vi "test_client.vi"() -> ()   [LabVIEW 2020]
uses:
  Client/Client.lvclass
  Request/Request.lvclass
  ClientBuilder/ClientBuilder.lvclass
  RequestBuilder/RequestBuilder.lvclass
  Types/http_method_enum.ctl
  reqwest.lvlib
  Headers/Headers.lvclass
panel:
  out "client_builder_error":string
  out "request_builder_error":string
  out "status code":u16
  out "response error":string
  out "has_response_error":bool
  in  "auth token":string
  in  "username":string
  in  "password":string
  out "response header":cluster{"header":string, "value":string}[](array[cluster])
  in  "file":path
  out "is_complete":bool
  out "progress":i32
  in  "abort":bool
  out "success":bool
  out "response body":string
  out "error out":errorcluster
  in  "url":string="https://www.vipm.io"
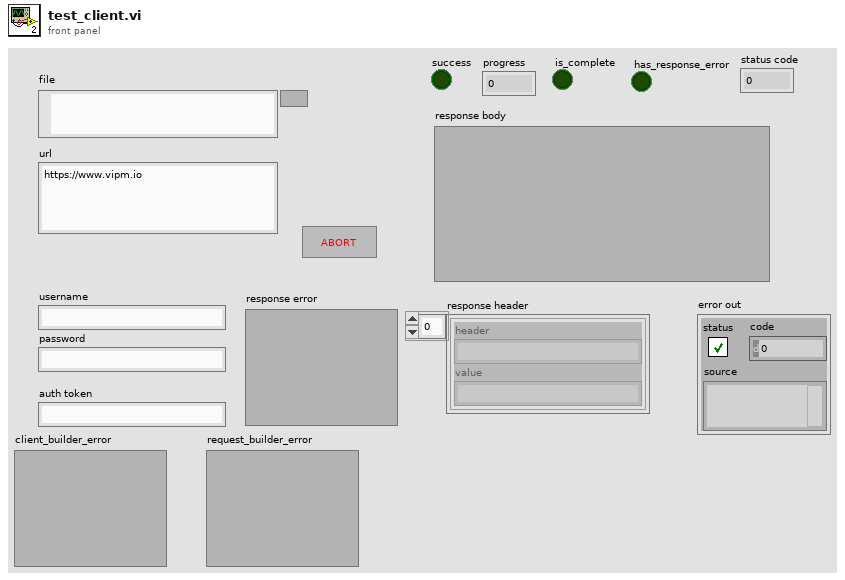
[diagram p1: front panel]
types:
  T1 = typedef "reqwest.lvlib/http_method_enum.ctl" = enum8{"<select>", "GET", "POST", "PUT", "DELETE", "HEAD", "OPTIONS", "CONNECT", "PATCH", "TRACE"}
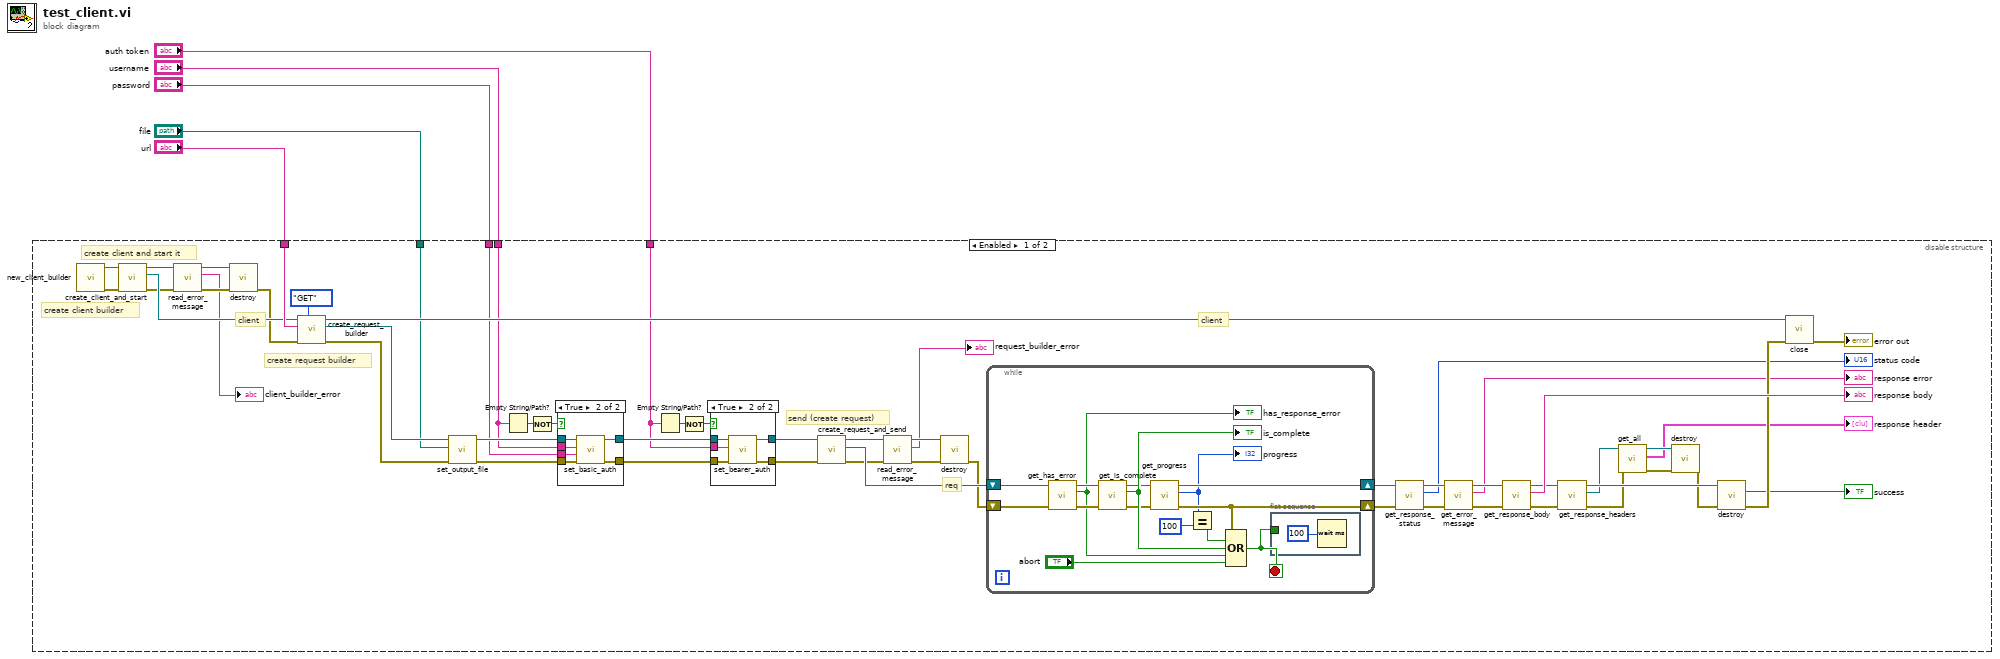
[diagram p0: block diagram]
diagram:
  n1 = disable-structure shown="Enabled" {
    disable-tunnel: "url" -> [w55 _]
    disable-tunnel: "file" -> [w49 _]
    disable-tunnel: "username" -> [w35 _]
    disable-tunnel: "password" -> [w34 _]
    disable-tunnel: "auth token" -> [w29 _]
    frame Enabled {
      # "send (create request)"
      # "create client builder"
      # "client"
      # "create client and start it"
      # "req"
      # "create request builder"
      # "client"
      n2 = call "new_client_builder.vi"() -> ("error out"=w56:errorcluster, "Client out"=w57:refnum<class "ClientBuilder.lvclass">)  [unwired: 10 in]
      n3 = call "create_client_and_start.vi"("error in"=w56, "ClientBuilder in"=w57) -> ("error out"=w8:errorcluster, "Client out"=w54:refnum<class "Client.lvclass">, "ClientBuilder out"=w11:refnum<class "ClientBuilder.lvclass">)  [unwired: 7 in]
      n4 = call "read_error_message.vi"("error in (no error)"=w8, "ClientBuilder in"=w11) -> ("error out"=w7:errorcluster, "error_message"=→"client_builder_error":string, "ClientBuilder in"=w9:refnum<class "ClientBuilder.lvclass">)  [unwired: 7 in]
      n5 = call "destroy.vi"("error in (no error)"=w7, "ClientBuilder in"=w9) -> ("error out"=w10:errorcluster)  [unwired: 9 in]
      n6 = call "create_request_builder.vi"("HTTP Method"=http_method_enum."GET", "error in (no error)"=w10, "url"=w55, "Client in"=w54) -> ("error out"=w51:errorcluster, "RequestBuilder out"=w52:refnum<class "RequestBuilder.lvclass">, "Client out"=w53:refnum<class "Client.lvclass">)  [unwired: 5 in]
      n7 = call "set_output_file.vi"("error in (no error)"=w51, "output_file"=w49, "obj in"=w52) -> ("error out"=w38:errorcluster, "obj out"=w39:refnum<class "RequestBuilder.lvclass">)  [unwired: 6 in, 1 out]
      n8 = Empty String/Path?(string/path=w35) -> (empty?=w37:bool)
      n9 = Not(x=w37) -> (.not. x?=w36:bool)
      n10 = case shown="True" w36 {
        tunnel: w39 -> [w70 w76]
        tunnel: [w70 w75] -> w31
        tunnel: w38 -> [w69 w74]
        tunnel: [w69 w73] -> w30
        tunnel: w35 -> [_ w72]
        tunnel: w34 -> [_ w71]
        frame False {
        }
        frame True {
          n11 = call "set_basic_auth.vi"("error in"=w74, "password"=w71, "username"=w72, "obj in"=w76) -> ("error out"=w73:errorcluster, "obj out"=w75:refnum<class "RequestBuilder.lvclass">)  [unwired: 5 in, 1 out]
        }
      }
      n12 = Empty String/Path?(string/path=w29) -> (empty?=w32:bool)
      n13 = Not(x=w32) -> (.not. x?=w33:bool)
      n14 = case shown="True" w33 {
        tunnel: w31 -> [w63 w68]
        tunnel: [w63 w67] -> w28
        tunnel: w30 -> [w62 w66]
        tunnel: [w62 w65] -> w27
        tunnel: w29 -> [_ w64]
        frame False {
        }
        frame True {
          n15 = call "set_bearer_auth.vi"("error in"=w66, "token"=w64, "obj in"=w68) -> ("error out"=w65:errorcluster, "obj out"=w67:refnum<class "RequestBuilder.lvclass">)  [unwired: 6 in, 1 out]
        }
      }
      n16 = call "create_request_and_send.vi"("error in"=w27, "obj in"=w28) -> ("error out"=w15:errorcluster, "request"=w18:refnum<class "Request.lvclass">, "obj out"=w16:refnum<class "RequestBuilder.lvclass">)  [unwired: 7 in]
      n17 = call "read_error_message.vi"("error in (no error)"=w15, "RequestBuilder in"=w16) -> ("error out"=w13:errorcluster, "error_message"=→"request_builder_error":string, "RequestBuilder in"=w17:refnum<class "RequestBuilder.lvclass">)  [unwired: 7 in]
      n18 = call "destroy.vi"("error in"=w13, "RequestBuilder in"=w17) -> ("error out"=w14:errorcluster)  [unwired: 8 in, 1 out]
      n19 = while {
        shift-right: [w88] -> w23
        shift-left: w18 -> [w81]
        shift-right: [w86] -> w22
        shift-left: w14 -> [w80]
        stop <- w82 stop-if-true
        n20 = call "get_has_error.vi"("error in (no error)"=w80, "Request in"=w81) -> ("error out"=w78:errorcluster, "has_error"=w77:bool, "Request out"=w79:refnum<class "Request.lvclass">)  [unwired: 7 in]
        "has_response_error" <- w77
        n21 = call "get_is_complete.vi"("error in (no error)"=w78, "Request in"=w79) -> ("error out"=w87:errorcluster, "is_complete"=w91:bool, "Request out"=w89:refnum<class "Request.lvclass">)  [unwired: 7 in]
        "is_complete" <- w91
        n22 = call "get_progress.vi"("error in (no error)"=w87, "Request in"=w89) -> ("error out"=w86:errorcluster, "progress"=w84:i32, "Request out"=w88:refnum<class "Request.lvclass">)  [unwired: 7 in]
        "progress" <- w84
        n23 = Equal?(x=w84, y=100 ("progress")) -> (x = y?=w83:bool)
        n24 = Compound Arithmetic op=OR(w86, w83, w91, w77, "abort") -> (w82:bool)
        n25 = flat-sequence {
          tunnel: w82 -> [_]
          frame #0 {
            n26 = Wait (ms)(milliseconds to wait=u32 100) -> ()  [unwired: 1 out]
          }
        }
      }
      n27 = call "get_response_status.vi"("error in (no error)"=w22, "Request in"=w23) -> ("error out"=w21:errorcluster, "status_code"=→"status code":u16, "Request out"=w20:refnum<class "Request.lvclass">)  [unwired: 7 in]
      n28 = call "get_error_message.vi"("error in (no error)"=w21, "Request in"=w20) -> ("error out"=w25:errorcluster, "error_message"=→"response error":string, "Request in"=w26:refnum<class "Request.lvclass">)  [unwired: 7 in]
      n29 = call "get_response_body.vi"("error in (no error)"=w25, "Request in"=w26) -> ("error out"=w46:errorcluster, "string_value"=→"response body":string, "Request in"=w48:refnum<class "Request.lvclass">)  [unwired: 7 in]
      n30 = call "get_response_headers.vi"("error in (no error)"=w46, "Request in"=w48) -> ("error out"=w44:errorcluster, "response_headers"=w45:refnum<class "Headers.lvclass">, "Request in"=w47:refnum<class "Request.lvclass">)  [unwired: 7 in]
      n31 = call "get_all.vi"("error in (no error)"=w44, "Headers in"=w45) -> ("error out"=w42:errorcluster, "headers"=→"response header":cluster{"name":string, "value":string}[], "Headers in"=w43:refnum<class "Headers.lvclass">)  [unwired: 6 in, 1 out]
      n32 = call "destroy.vi"("error in (no error)"=w42, "Headers in"=w43) -> ("error out"=w41:errorcluster)  [unwired: 9 in]
      n33 = call "destroy.vi"("error in (no error)"=w41, "Request in"=w47) -> ("error out"=w59:errorcluster, "success"=→"success":bool)  [unwired: 8 in]
      n34 = call "close.vi"("error in (no error)"=w59, "Client in"=w53) -> ("error out"=→"error out":errorcluster)  [unwired: 9 in]
    }
    frame Disabled {
    }
  }
